vi "UI Subpanel.vi"() -> ()   [LabVIEW 2021, in "CIF CAN_Writer_NIXNET UI.lvlib"]
uses:
  CIF CAN_Writer_NIXNET UI.lvlib
  Common/Typedef/Configuration.ctl
  <vilib>/CIF Foundation/CIF Core/CIFCore/Common/Typedef/Common Plugin Configuration.ctl
  <vilib>/CIF Foundation/CIF Core/CIFCore/Common/Typedef/External Clock Config.ctl
  <vilib>/CIF Foundation/CIF CAN RW Core/typedef/CAN Port Configuration.ctl
  <vilib>/CIF Foundation/CIF CAN RW Core/typedef/CAN Mode.ctl
  <vilib>/CIF Foundation/CIF CAN RW Core/typedef/FD Config.ctl
  <vilib>/CIF Foundation/CIF CAN RW Core/typedef/CAN Filter.ctl
  <vilib>/CIF Foundation/CIF Core/CIFUI/Typedef/Class Data for SubPanel.ctl
  <vilib>/CIF Foundation/CIF Core/CIFUI/Typedef/Core UI References.ctl
  <vilib>/CIF Foundation/CIF Core/CIFUI/Typedef/Run Listen Button.ctl
  <vilib>/CIF Foundation/CIF Core/CIFUI/Typedef/SubPanel Events.ctl
  <vilib>/CIF Foundation/CIF Core/CIFUI/Typedef/New Connection Plugin Event Data.ctl
  Grpc/CanWriterNixnet_client/RPC Messages/cif_can_writer_nixnet_Statistics.ctl
  Typedef/UI CAN Message Input.ctl
  <vilib>/xnet/xnet.llb/XNET Frame Type CAN.ctl
  <vilib>/CIF Foundation/CIF Core/CIFCore/Common/Typedef/FIFO Statistics.ctl
  <vilib>/CIF Foundation/CIF Core/CIFCore/Common/Typedef/Timing Stats Base.ctl
  <vilib>/CIF Foundation/CIF CAN RW Core/typedef/CAN Status.ctl
  <vilib>/CIF Foundation/CIF CAN RW Core/typedef/Communication State.ctl
  <vilib>/CIF Foundation/CIF CAN RW Core/typedef/Last Error.ctl
  <vilib>/CIF Foundation/CIF Core/CIFUI/CIF_UI.lvclass
  <vilib>/CIF Foundation/CIF Core/CIFUI/CIF_UI.lvclass/CIF_UI.ctl
  <vilib>/CIF Foundation/CIF XNET CAN RW/XNET CAN RW.lvclass
  <vilib>/xnet/xnet.llb/XNET Frame CAN.ctl
  <vilib>/CIF Foundation/CIF Core/CIFUI/Utilities/Get Human Readable Error.vi
  <vilib>/CIF Foundation/CIF Utilities/Errors/Append Error Location.vi
  <vilib>/CIF Foundation/CIF Utilities/Errors/Human Readable Error Message.vi
  Grpc/CAN_Writer_NIXNET_wrapper/CAN_Writer_NIXNET_Wrapper.lvlib
  <vilib>/addons/_JKI.lib/Serialization/JSON/JKI JSON Serialization.lvlib
  <vilib>/CIF Foundation/CIF Core/CIFCore/Grpc/CIFCoreWrapper/CIFCoreWrapper.lvlib
  <vilib>/CIF Foundation/CIF Core/CIFCore/Common/CIFCoreCommon.lvlib
  Common/CAN_Writer_NIXNET_Common.lvlib
  <vilib>/CIF Foundation/CIF CAN RW Core/CAN_RW_CORE.lvclass
  Grpc/CanWriterNixnet_client/CanWriterNixnet_client.lvlib
panel:
  out "CAN Status":T1
  out "FIFO Statistics (us)":T4
  in  "CAN Messages to Send":T6[](array[typedef]) {"type" items=["CAN Data"=0, "CAN Remote"=1, "CAN Bus Error"=2, "CAN 2.0 Data"=8, "CAN FD Data"=16, "CAN FD+BRS Data"=24, "J1939 Data"=192, "Delay"=224, "Log Trigger"=225, "Start Trigger"=226]; "identifier" format="%x"}
  in  "Send CAN Message":bool
  out "Statistics":T8
  out "Devices":string[](array[string])
  in  "Blink":bool
  in  "Refresh Device List":bool
  in  "Class Data for SubPanel":T9
  in  "Update Config":bool
  in  "Configuration":T12={"Common"={"Period (s)"=0.001, "Offset (us)"=0, "Priority"=100, "Processor"=-2, "External Clock"={"ClockID"=0, "Clock Name"="", "Publish Clock"=FALSE, "Convert Data Timestamps"=FALSE, "Plugin Timing Source"=FALSE}}, "TX Interface"="CAN2", "Port Configuration"={"Mode"=enum."CAN FD", "Baud Rate"=500000, "Temination On"=TRUE, "Subordinate"=FALSE, "Echo TX"=FALSE, "FD Config"={"FD Baud Rate"=2000000, "ISO Mode"=TRUE, "BRS Enabled"=TRUE}}, "Filter"={"Allow List (ID)"=[], "Deny List (ID)"=[]}, "Wake Offset (us)"=100, "One Shot"=FALSE} {"Filter"."Deny List (ID)" format="%.0x"; "Filter"."Allow List (ID)" format="%.0x"; "Port Configuration"."FD Config"."FD Baud Rate" format="%.0p"; "Port Configuration"."Baud Rate" format="%.0p"; "Common"."Period (s)" format="%#_13g"}
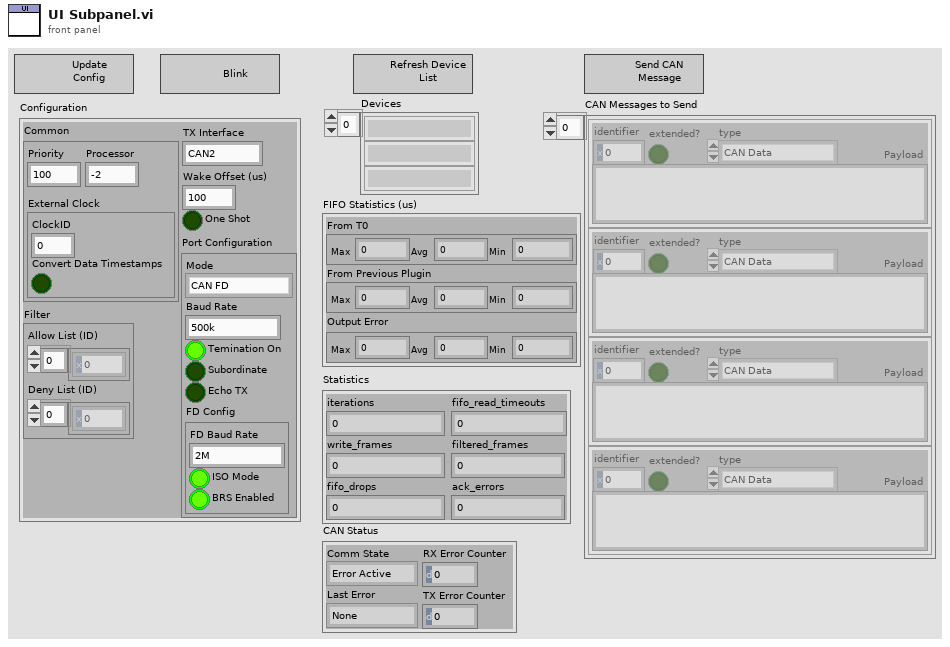
[diagram p1: front panel]
types:
  T1 = typedef "CAN_RW_CORE.lvclass/CAN Status.ctl" = cluster{"Comm State":T2, "Last Error":T3, "RX Error Counter":u8, "TX Error Counter":u8}
  T2 = typedef "CAN_RW_CORE.lvclass/Communication State.ctl" = enum16{"Error Active", "Error Passive", "Bus Off"}
  T3 = typedef "CAN_RW_CORE.lvclass/Last Error.ctl" = enum16{"None", "Stuff", "Form", "Ack", "Bit1", "Bit0", "CRC", "Unknown"}
  T4 = typedef "CIFCoreCommon.lvlib/FIFO Statistics.ctl" = cluster{"From T0":T5, "From Previous Plugin":T5, "Output Error":T5}
  T5 = typedef "CIFCoreCommon.lvlib/Timing Stats Base.ctl" = cluster{"Max":i64, "Avg":dbl, "Min":i64}
  T6 = typedef "CIF CAN_Writer_NIXNET UI.lvlib/UI CAN Message Input.ctl" = cluster{"identifier":u32, "extended?":bool, "type":T7, "Payload":string}
  T7 = typedef "XNET Frame Type CAN.ctl" = u8
  T8 = typedef "CanWriterNixnet_client.lvlib/cif_can_writer_nixnet_Statistics.ctl" = cluster{"iterations":u64, "fifo_read_timeouts":u64, "write_frames":u64, "filtered_frames":u64, "fifo_drops":u64, "ack_errors":u64}
  T9 = typedef "CIF_UI.lvclass/Class Data for SubPanel.ctl" = cluster{"IP Address":string, "Server Certificate File (.crt)":path, "Connected":bool, "Core UI References":T10, "Subpanel Events":T11, "Manager gRPC Port":u16}
  T10 = typedef "CIF_UI.lvclass/Core UI References.ctl" = cluster{"Plugin Status":refnum<vi>, "Plugin Status Valid":bool, "Connection":refnum<vi>, "Connection Valid":bool, "Exit":refnum<vi>, "Exit Valid":bool, "Run Listen":refnum<vi>, "Run Listen Valid":bool, "Clear Local Error":refnum<vi>, "Clear Local Error Valid":bool, "Local Error":refnum<vi>, "Local Error Valid":bool}
  T11 = typedef "CIF_UI.lvclass/SubPanel Events.ctl" = cluster{"Clear Local Error":refnum<user-event>, "Shutdown":refnum<user-event>, "Plugin Connection":refnum<user-event>}
  T12 = typedef "CAN_Writer_NIXNET_Common.lvlib/Configuration.ctl" = cluster{"Common":T13, "TX Interface":string, "Port Configuration":T15, "Filter":T18, "Wake Offset (us)":i64, "One Shot":bool}
  T13 = typedef "CIFCoreCommon.lvlib/Common Plugin Configuration.ctl" = cluster{"Period (s)":dbl, "Offset (us)":i32, "Priority":i32, "Processor":i32, "External Clock":T14}
  T14 = typedef "CIFCoreCommon.lvlib/External Clock Config.ctl" = cluster{"ClockID":u8, "Clock Name":string, "Publish Clock":bool, "Convert Data Timestamps":bool, "Plugin Timing Source":bool}
  T15 = typedef "CAN_RW_CORE.lvclass/CAN Port Configuration.ctl" = cluster{"Mode":T16, "Baud Rate":u64, "Temination On":bool, "Subordinate":bool, "Echo TX":bool, "FD Config":T17}
  T16 = typedef "CAN_RW_CORE.lvclass/CAN Mode.ctl" = enum16{"CAN 2.0", "CAN FD"}
  T17 = typedef "CAN_RW_CORE.lvclass/FD Config.ctl" = cluster{"FD Baud Rate":u64, "ISO Mode":bool, "BRS Enabled":bool}
  T18 = typedef "CAN_RW_CORE.lvclass/CAN Filter.ctl" = cluster{"Allow List (ID)":u32[], "Deny List (ID)":u32[]}
  T19 = typedef "grpc-lvsupport-release.lvlib/grpcId.ctl" = u64
  T20 = typedef "XNET Frame CAN.ctl" = cluster{"timestamp":timestamp, "payload":u8[], "identifier":u32, "type":T7, "extended?":bool, "echo?":bool}
  T21 = typedef "CIFCoreCommon.lvlib/gRPC Reported Plugin Status.ctl" = cluster{"State":T22, "Timing Statistics (us)":T23, "FIFO Statistics (us)":T4, "error":T24, "Monitor Doubles":T25, "Monitor U64":T26, "Monitor I64":T27}
  T22 = typedef "CIFCoreCommon.lvlib/Plugin State.ctl" = enum8{"Null", "Creating", "Listening", "Running", "CleaningUp", "Destroying", "Prepared", "FTE_Run"}
  T23 = typedef "CIFCoreCommon.lvlib/Timing Statistics.ctl" = cluster{"Period":T5, "Wake Error":T5, "Execute":T5, "Housekeep":T5, "Idle":T5, "Cleanup":T5, "Custom 1 (custom units)":T5, "Custom 2 (custom units)":T5}
  T24 = typedef "CIFCoreCommon.lvlib/Simple Error.ctl" = cluster{"status":bool, "code":i32}
  T25 = typedef "CIFCoreCommon.lvlib/Monitor Doubles.ctl" = cluster{"1":dbl, "2":dbl, "3":dbl, "4":dbl}
  T26 = typedef "CIFCoreCommon.lvlib/Monitor U64.ctl" = cluster{"1":u64, "2":u64, "3":u64, "4":u64}
  T27 = typedef "CIFCoreCommon.lvlib/Monitor I64.ctl" = cluster{"1":i64, "2":i64, "3":i64, "4":i64}
  T28 = typedef "CanWriterNixnet_client.lvlib/cif_can_writer_nixnet_XnetDevice.ctl" = cluster{"interface":string, "slot":u32, "device_id":string}
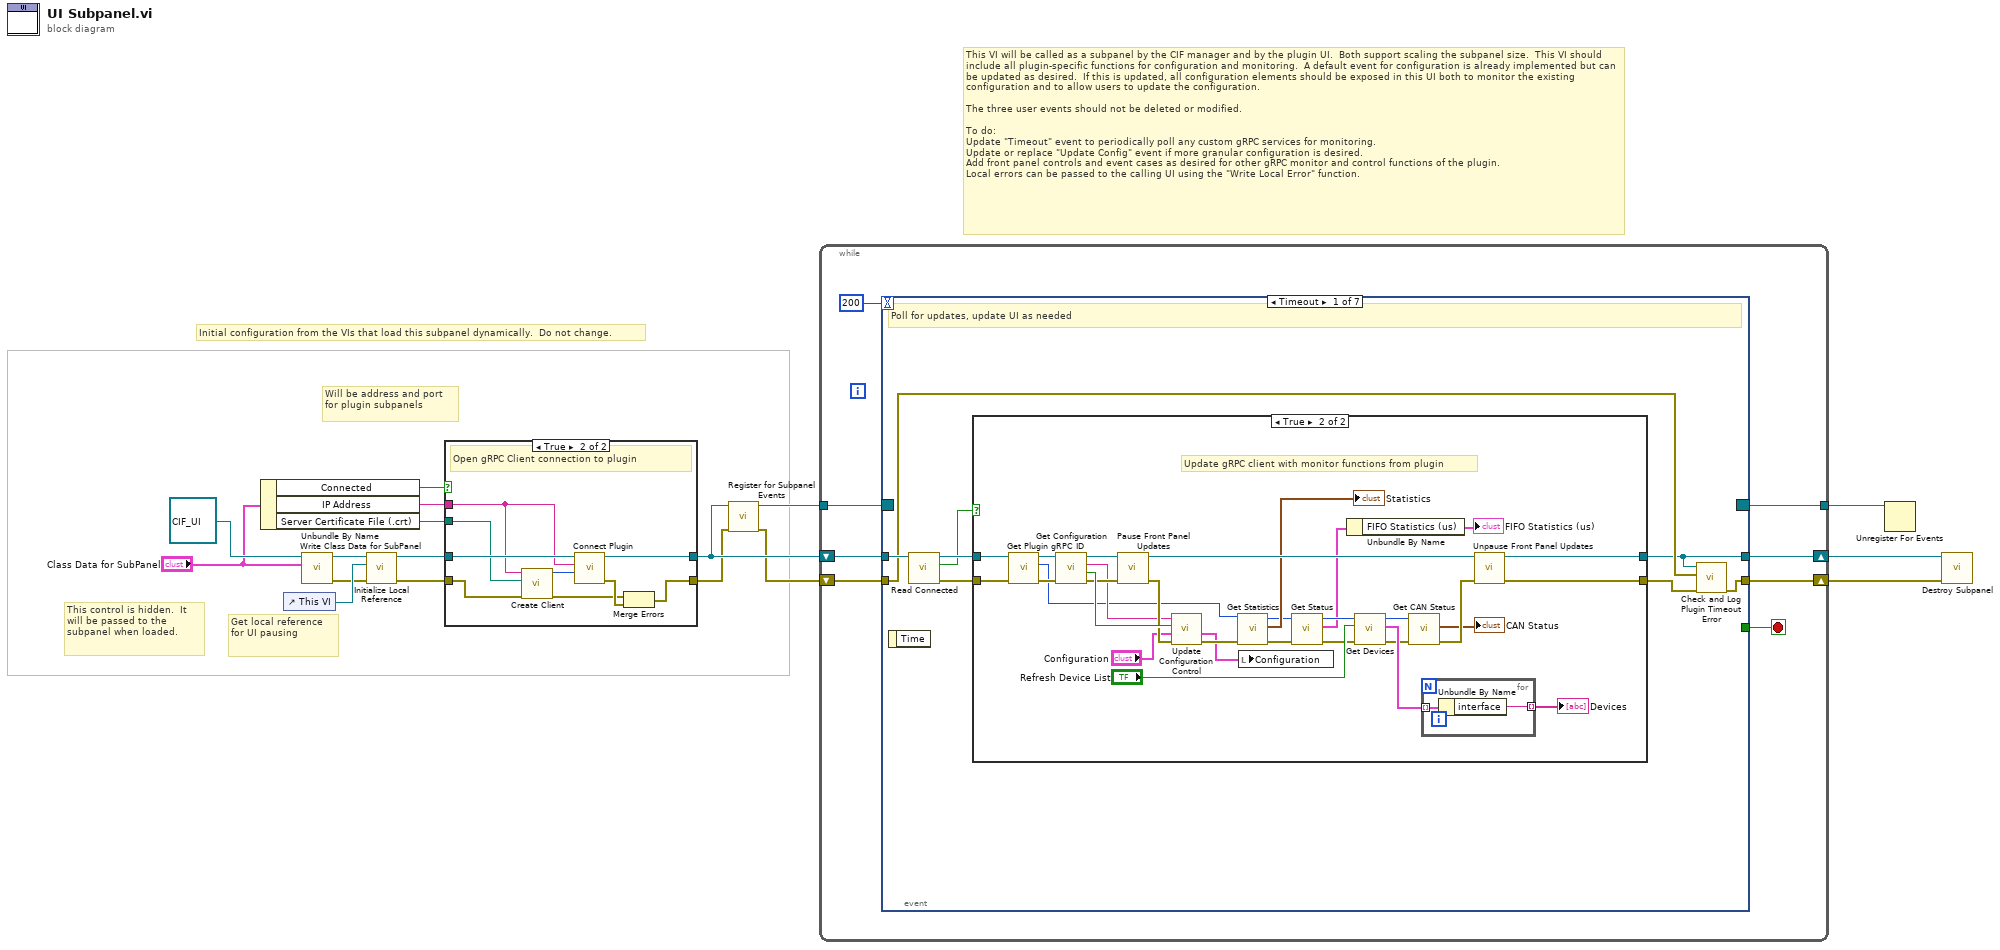
[diagram p0: block diagram]
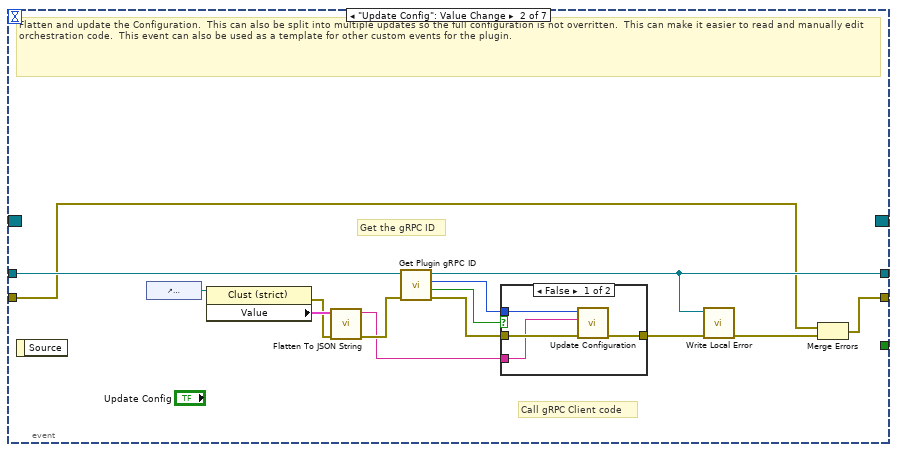
[diagram p4: hidden frame]
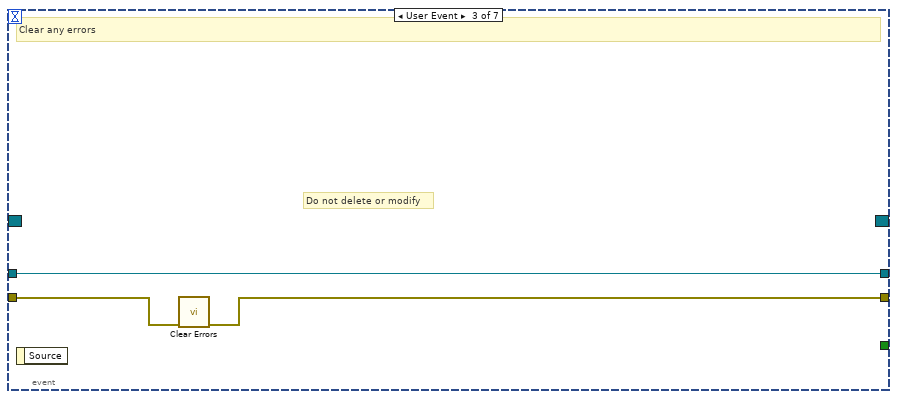
[diagram p6: hidden frame]
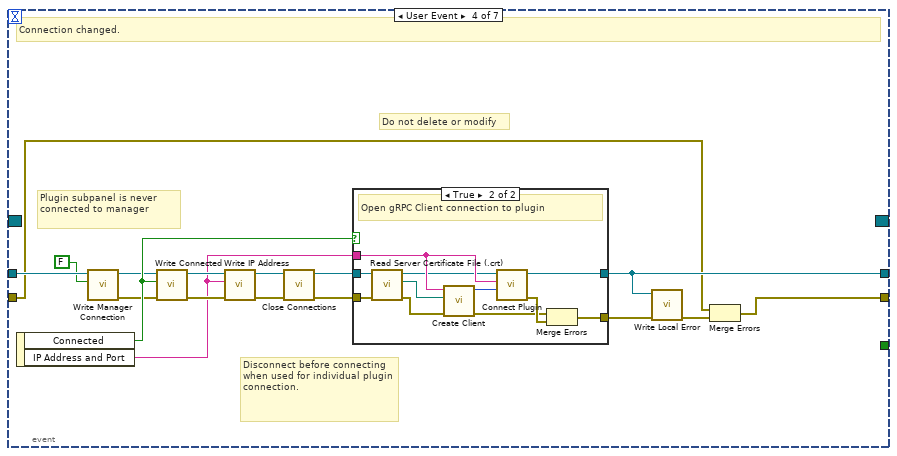
[diagram p7: hidden frame]
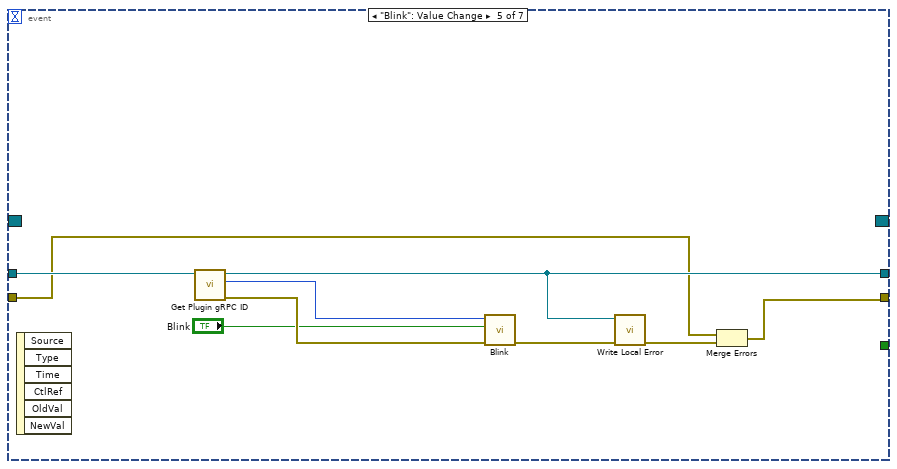
[diagram p9: hidden frame]
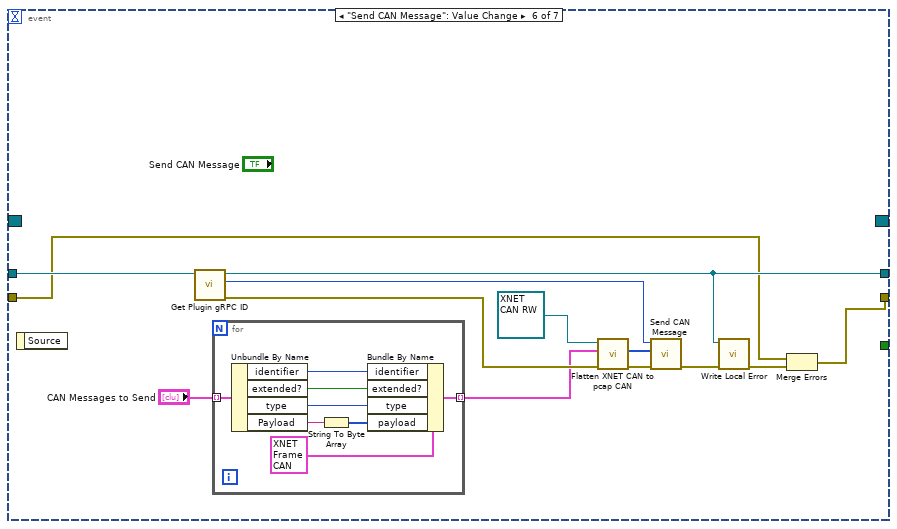
[diagram p10: hidden frame]
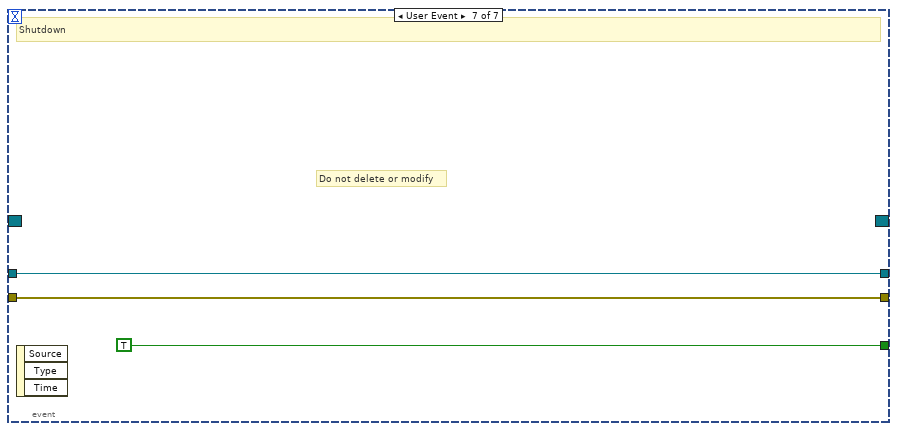
[diagram p11: hidden frame]
diagram:
  # "Initial configuration from the VIs that load this subpanel dynamically.  Do not change."
  # "This control is hidden.  It will be passed to the subpanel when loaded."
  # "This VI will be called as a subpanel by the CIF manager and by the plugin UI.  Both support scaling the subpanel size.  This VI should include all plugin-specific functions for configuration and monitoring.  A default event for configuration is already implemented but can be updated as desired.  If this is updated, all configuration elements should be exposed in this UI both to monitor the existing configuration and to allow users to update the configuration.\n\nThe three user events should not be deleted or modified.\n\nTo do:\nUpdate \"Timeout\" event to periodically poll any custom gRPC services for monitoring.\nUpdate or replace \"Update Config\" event if more granular configuration is desired.\nAdd front panel controls and event cases as desired for other gRPC monitor and control functions of the plugin.\nLocal errors can be passed to the calling UI using the \"Write Local Error\" function."
  # "Will be address and port for plugin subpanels"
  # "Get local reference for UI pausing"
  n1 = Unbundle By Name("Class Data for SubPanel") -> ("Connected"=w8:bool, "IP Address"=w7:string, "Server Certificate File (.crt)"=w6:path)
  n2 = control-ref of="This VI"() -> (w17:refnum<vi>)
  n3 = call <vilib>:"Write Class Data for SubPanel.vi"("Class Data for SubPanel"="Class Data for SubPanel", "CIF_UI in"=refnum<class "CIF_UI.lvclass"> refnum) -> ("error out"=w12:errorcluster, "CIF_UI out"=w14:refnum<class "CIF_UI.lvclass">)  [unwired: 8 in]
  n4 = call <vilib>:"Initialize Local Reference.vi"("error in (no error)"=w12, "This VI"=w17, "CIF_UI in"=w14) -> ("error out"=w10:errorcluster, "CIF_UI out"=w11:refnum<class "CIF_UI.lvclass">)  [unwired: 7 in]
  n5 = case shown="True" w8 {
    tunnel: [w18 w28] -> w4
    tunnel: [w19 w26] -> w5
    tunnel: w11 -> [w19 w25]
    tunnel: w10 -> [w18 w24]
    tunnel: w7 -> [_ w21]
    tunnel: w6 -> [_ w20]
    frame False {
    }
    frame True {
      # "Open gRPC Client connection to plugin"
      n6 = call "Create Client.vi"("error in"=w24, "Server Certificate File (.crt)"=w20, "address"=w21) -> ("error out"=w23:errorcluster, "gRPC ID Out"=w22:T19)  [unwired: 7 in]
      n7 = call <vilib>:"Connect Plugin.vi"("gRPC ID"=w22, "Address"=w21, "CIF_UI in"=w25) -> ("error out"=w27:errorcluster, "CIF_UI out"=w26:refnum<class "CIF_UI.lvclass">)  [unwired: 7 in]
      n8 = Merge Errors(w23, w27) -> (w28:errorcluster)
    }
  }
  n9 = call <vilib>:"Register for Subpanel Events.vi"("error in (no error)"=w4, "CIF_UI in"=w5) -> ("error out"=w2:errorcluster, "Event Registration Refnum"=w3:refnum<event-registration>)  [unwired: 8 in]
  n10 = while {
    tunnel: w3 -> [w35]
    shift-right: [w30] -> w16
    shift-left: w5 -> [w33]
    shift-right: [w31] -> w1
    shift-left: w2 -> [w32]
    tunnel: [w29] -> w15
    stop <- w34 stop-if-true
    n11 = event shown="[0] Timeout" {
      selector: w35 -> [_ _ _ _ _ _ _]
      dyn-events: [_ _ _ _ _ _ _] -> w29
      timeout: 200 -> [_ _ _ _ _ _ _]
      tunnel: [_ _ _ _ _ _ TRUE] -> w34
      tunnel: w33 -> [w41 w89 w98 w109 w138 w151 w162]
      tunnel: w32 -> [w38 w83 w100 w102 w133 w147 w161]
      tunnel: [w39 w82 w99 w101 w132 w146 w161] -> w31
      tunnel: [w37 w85 w98 w103 w135 w149 w162] -> w30
      event Timeout {
        # "Poll for updates, update UI as needed"
        n12 = event-data() -> ()  [unwired: 1 in, 1 out]
        n13 = call <vilib>:"Read Connected.vi"("CIF_UI in"=w41) -> ("error out"=w43:errorcluster, "Connected"=w42:bool, "CIF_UI out"=w44:refnum<class "CIF_UI.lvclass">)  [unwired: 8 in]
        n14 = case shown="True" w42 {
          tunnel: w43 -> [w45 w68]
          tunnel: [w45 w76] -> w40
          tunnel: w44 -> [w46 w69]
          tunnel: [w46 w75] -> w37
          frame False {
          }
          frame True {
            # "Update gRPC client with monitor functions from plugin"
            n15 = call <vilib>:"Get Plugin gRPC ID.vi"("error in (no error)"=w68, "CIF_UI in"=w69) -> ("error out"=w66:errorcluster, "gRPC ID"=w63:T19, "CIF_UI out"=w67:refnum<class "CIF_UI.lvclass">)  [unwired: 5 in, 2 out]
            n16 = call <vilib>:"Get Configuration.vi"("error in (no error)"=w66, "CIF_Plugin_UI in"=w67) -> ("error out"=w72:errorcluster, "Not Found"=w74:bool, "JSON Configuration"=w65:string, "CIF_Plugin_UI out"=w73:refnum<class "CIF_UI.lvclass">)  [unwired: 6 in]
            n17 = call <vilib>:"Pause Front Panel Updates.vi"("error in (no error)"=w72, "CIF_UI in"=w73) -> ("error out"=w71:errorcluster, "CIF_UI out"=w70:refnum<class "CIF_UI.lvclass">)  [unwired: 8 in]
            n18 = call "Update Configuration Control.vi"("error in (no error)"=w71, "Configuration in"="Configuration", "Not Valid"=w74, "JSON Configuration"=w65) -> ("error out"=w64:errorcluster, "Configuration out"=w61:T12)  [unwired: 6 in]
            n19 = call "Get Statistics.vi"("error in"=w64, "gRPC ID"=w63) -> ("error out"=w55:errorcluster, "Statistics"=→"Statistics":T8, "gRPC ID out"=w56:T19)  [unwired: 7 in]
            n20 = local write "Configuration"(w61) -> ()
            n21 = call <vilib>:"Get Status.vi"("error in"=w55, "gRPC ID"=w56) -> ("error out"=w54:errorcluster, "Node Status"=w52:T21, "gRPC ID out"=w53:T19)  [unwired: 7 in]
            n22 = Unbundle By Name(w52) -> ("FIFO Statistics (us)"=→"FIFO Statistics (us)":T4)
            n23 = call "Get Devices.vi"("error in"=w54, "Refresh Device List"="Refresh Device List", "gRPC ID"=w53) -> ("error out"=w50:errorcluster, "devices"=w58:T28[], "gRPC ID out"=w48:T19)  [unwired: 6 in]
            n24 = call "Get CAN Status.vi"("error in"=w50, "gRPC ID"=w48) -> ("error out"=w49:errorcluster, "CAN Status"=→"CAN Status":T1)  [unwired: 7 in, 1 out]
            n25 = for {
              tunnel: w58 -> [w78] mode=indexing
              tunnel: [w77] -> w59 mode=indexing
              n26 = Unbundle By Name(w78) -> ("interface"=w77:string)
            }
            "Devices" <- w59
            n27 = call <vilib>:"Unpause Front Panel Updates.vi"("error in (no error)"=w49, "CIF_UI in"=w70) -> ("error out"=w76:errorcluster, "CIF_UI out"=w75:refnum<class "CIF_UI.lvclass">)  [unwired: 8 in]
          }
        }
        n28 = call <vilib>:"Check and Log Plugin Timeout Error.vi"("New Error"=w40, "Previous Error"=w38, "CIF_UI in"=w37) -> ("error out"=w39:errorcluster)  [unwired: 8 in]
      }
      event "Update Config": Value Change {
        # "Call gRPC Client code"
        # "Get the gRPC ID"
        # "Flatten and update the Configuration.  This can also be split into multiple updates so the full configuration is not overritten.  This can make it easier to read and manually edit orchestration code.  This event can also be used as a template for other custom events for the plugin."
        n29 = event-data() -> ()  [unwired: 1 in, 1 out]
        n30 = control-ref of="Configuration"() -> (w81:refnum<vi>)
        n31 = property class="Clust (strict)"(reference=w81) -> (error out=w79:errorcluster, "Value"=w80:T12)  [unwired: 1 in, 1 out]
        n32 = call <vilib>:"Flatten To JSON String.vi"("error in"=w79, "Variant"=w80) -> ("error out"=w88:errorcluster, "JSON String"=w87:string)  [unwired: 8 in]
        n33 = call <vilib>:"Get Plugin gRPC ID.vi"("error in (no error)"=w88, "CIF_UI in"=w89) -> ("error out"=w90:errorcluster, "Not Found"=w91:bool, "gRPC ID"=w92:T19, "CIF_UI out"=w85:refnum<class "CIF_UI.lvclass">)  [unwired: 5 in, 1 out]
        n34 = case shown="False" w91 {
          tunnel: w92 -> [w96 _]
          tunnel: w90 -> [w95 w97]
          tunnel: [w94 w97] -> w86
          tunnel: w87 -> [w93 _]
          frame False {
            n35 = call <vilib>:"Update Configuration.vi"("error in"=w95, "JSON Configuration"=w93, "gRPC ID"=w96) -> ("error out"=w94:errorcluster)  [unwired: 7 in, 1 out]
          }
          frame True {
          }
        }
        n36 = call <vilib>:"Write Local Error.vi"("error in (no error)"=w86, "CIF_UI in"=w85) -> ("error out"=w84:errorcluster)  [unwired: 9 in]
        n37 = Merge Errors(w83, w84) -> (w82:errorcluster)
      }
      event User Event {
        # "Do not delete or modify"
        # "Clear any errors"
        n38 = event-data() -> ()  [unwired: 1 in, 1 out]
        n39 = call <vilib>:"Clear Errors.vi"("error in (no error)"=w100) -> ("error out"=w99:errorcluster)  [unwired: 5 in, 1 out]
      }
      event User Event {
        # "Do not delete or modify"
        # "Plugin subpanel is never connected to manager"
        # "Disconnect before connecting when used for individual plugin connection."
        # "Connection changed."
        n40 = event-data() -> ("Connected"=w110:bool, "IP Address and Port"=w111:string)  [unwired: 1 in]
        n41 = call <vilib>:"Write Manager Connection.vi"("Manager Connection"=FALSE, "CIF_UI in"=w109) -> ("error out"=w107:errorcluster, "CIF_UI out"=w108:refnum<class "CIF_UI.lvclass">)  [unwired: 8 in]
        n42 = call <vilib>:"Write Connected.vi"("error in (no error)"=w107, "Connected"=w110, "CIF_UI in"=w108) -> ("error out"=w116:errorcluster, "CIF_UI out"=w117:refnum<class "CIF_UI.lvclass">)  [unwired: 7 in]
        n43 = call <vilib>:"Write IP Address.vi"("error in (no error)"=w116, "IP Address"=w111, "CIF_UI in"=w117) -> ("error out"=w114:errorcluster, "CIF_UI out"=w115:refnum<class "CIF_UI.lvclass">)  [unwired: 7 in]
        n44 = call <vilib>:"Close Connections.vi"("error in (no error)"=w114, "CIF_UI in"=w115) -> ("error out"=w112:errorcluster, "CIF_UI out"=w113:refnum<class "CIF_UI.lvclass">)  [unwired: 8 in]
        n45 = case shown="True" w110 {
          tunnel: [w118 w130] -> w104
          tunnel: [w119 w128] -> w103
          tunnel: w113 -> [w119 w124]
          tunnel: w112 -> [w118 w123]
          tunnel: w111 -> [_ w125]
          frame False {
          }
          frame True {
            # "Open gRPC Client connection to plugin"
            n46 = call <vilib>:"Read Server Certificate File (.crt).vi"("error in (no error)"=w123, "CIF_UI in"=w124) -> ("error out"=w121:errorcluster, "Server Certificate File (.crt)"=w120:path, "CIF_UI out"=w122:refnum<class "CIF_UI.lvclass">)  [unwired: 7 in]
            n47 = call "Create Client.vi"("error in"=w121, "Server Certificate File (.crt)"=w120, "address"=w125) -> ("error out"=w127:errorcluster, "gRPC ID Out"=w126:T19)  [unwired: 7 in]
            n48 = call <vilib>:"Connect Plugin.vi"("gRPC ID"=w126, "Address"=w125, "CIF_UI in"=w122) -> ("error out"=w129:errorcluster, "CIF_UI out"=w128:refnum<class "CIF_UI.lvclass">)  [unwired: 7 in]
            n49 = Merge Errors(w127, w129) -> (w130:errorcluster)
          }
        }
        n50 = call <vilib>:"Write Local Error.vi"("error in (no error)"=w104, "CIF_UI in"=w103) -> ("error out"=w105:errorcluster)  [unwired: 9 in]
        n51 = Merge Errors(w102, w105) -> (w101:errorcluster)
      }
      event "Blink": Value Change {
        n52 = event-data() -> ()  [unwired: 1 in, 6 out]
        n53 = call <vilib>:"Get Plugin gRPC ID.vi"("CIF_UI in"=w138) -> ("error out"=w137:errorcluster, "gRPC ID"=w136:T19, "CIF_UI out"=w135:refnum<class "CIF_UI.lvclass">)  [unwired: 6 in, 2 out]
        n54 = call "Blink.vi"("error in"=w137, "blink"="Blink", "gRPC ID"=w136) -> ("error out"=w134:errorcluster)  [unwired: 7 in, 1 out]
        n55 = call <vilib>:"Write Local Error.vi"("error in (no error)"=w134, "CIF_UI in"=w135) -> ("error out"=w139:errorcluster)  [unwired: 9 in]
        n56 = Merge Errors(w133, w139) -> (w132:errorcluster)
      }
      event "Send CAN Message": Value Change {
        n57 = event-data() -> ()  [unwired: 1 in, 1 out]
        n58 = call <vilib>:"Get Plugin gRPC ID.vi"("CIF_UI in"=w151) -> ("error out"=w144:errorcluster, "gRPC ID"=w150:T19, "CIF_UI out"=w149:refnum<class "CIF_UI.lvclass">)  [unwired: 6 in, 2 out]
        n59 = for {
          tunnel: "CAN Messages to Send" -> [w160] mode=indexing
          tunnel: [w153] -> w141 mode=indexing
          n60 = Unbundle By Name(w160) -> ("identifier"=w158:u32, "extended?"=w157:bool, "type"=w156:T7, "Payload"=w155:string)
          n61 = String To Byte Array(string=w155) -> (unsigned byte array=w154:u8[])
          n62 = Bundle By Name(cluster=T20 {"timestamp"=timestamp(0 s since 1904-01-01), "payload"=[], "identifier"=0, "type"=0, "extended?"=FALSE, "echo?"=FALSE} ("CAN frame"), "identifier"=w158, "extended?"=w157, "type"=w156, "payload"=w154) -> (w153:T20)
        }
        n63 = call <vilib>:"Flatten XNET CAN to pcap CAN.vi"("error in (no error)"=w144, "XNET CAN Data"=w141, "XNET_CAN_RW in"=refnum<class "XNET CAN RW.lvclass"> refnum ("CAN_Logic in")) -> ("error out"=w143:errorcluster, "pcap CAN DATA"=w140:u8[])  [unwired: 6 in, 1 out]
        n64 = call "Send CAN Message.vi"("error in"=w143, "CAN Message"=w140, "gRPC ID"=w150) -> ("error out"=w148:errorcluster)  [unwired: 7 in, 1 out]
        n65 = call <vilib>:"Write Local Error.vi"("error in (no error)"=w148, "CIF_UI in"=w149) -> ("error out"=w152:errorcluster)  [unwired: 9 in]
        n66 = Merge Errors(w147, w152) -> (w146:errorcluster)
      }
      event User Event {
        # "Do not delete or modify"
        # "Shutdown"
        n67 = event-data() -> ()  [unwired: 1 in, 3 out]
      }
    }
  }
  n68 = Unregister For Events(event registration refnum=w15) -> ()  [unwired: 1 in, 1 out]
  n69 = call <vilib>:"Destroy Subpanel.vi"("error in (no error)"=w1, "CIF_UI in"=w16) -> ()  [unwired: 8 in, 2 out]
